vi "Init.vi"(8 "error in (no error)":errorcluster, 10 "CONTROLLER":refnum<class "CONTROLLER.lvclass">, 11 "VIEW in":refnum<class "VIEW.lvclass">) -> (0 "error out":errorcluster, 3 "VIEW out":refnum<class "VIEW.lvclass">)   [LabVIEW 2013, in "VIEW.lvclass"]
uses:
  VIEW.lvclass
  Controller/base/CONTROLLER.lvclass
  VIEW.lvclass/VIEW.ctl
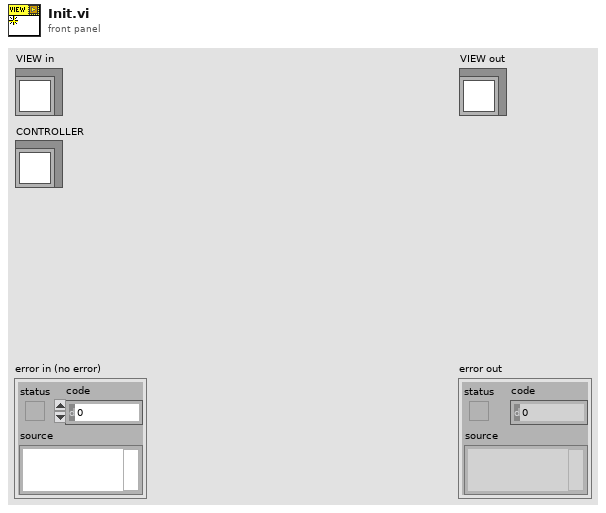
[diagram p1: front panel]
types:
  T1 = cluster{"CtlRef":refnum<vi>, "Name":string, "ClassName":string}
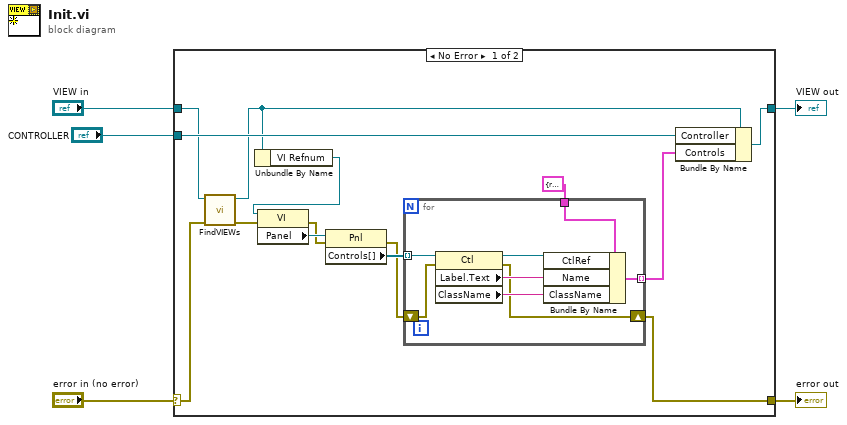
[diagram p0: block diagram]
diagram:
  n1 = case shown="No Error" "error in (no error)" {
    selector: "error in (no error)" -> [w10 w29]
    tunnel: [w13 w29] -> w4
    tunnel: [w12 w28] -> w2
    tunnel: "VIEW in" -> [w8 w28]
    tunnel: "CONTROLLER" -> [w11 _]
    frame No Error {
      n2 = call-dynamic "FindVIEWs.vi"("error in (no error)"=w10, "VIEW in"=w8) -> ("error out"=w9:errorcluster, "VIEW out"=w7:refnum<class "VIEW.lvclass">)  [unwired: 8 in]
      n3 = Unbundle By Name(w7) -> ("VI Refnum"=w6:refnum<vi>)
      n4 = property class="VI"(reference=w6, error in=w9) -> (error out=w18:errorcluster, "Panel"=w19:refnum<vi>)  [unwired: 1 out]
      n5 = property class="Pnl"(reference=w19, error in=w18) -> (error out=w14:errorcluster, "Controls[]"=w17:refnum<vi>[])  [unwired: 1 out]
      n6 = for {
        tunnel: w17 -> [w27] mode=indexing
        tunnel: T1 {"CtlRef"=refnum, "Name"="", "ClassName"=""} ("CtlInfo") -> [w26]
        tunnel: [w22] -> w15 mode=indexing
        shift-right: [w20] -> w13
        shift-left: w14 -> [w21]
        n7 = property class="Ctl"(reference=w27, error in=w21) -> (reference out=w25:refnum<vi>, error out=w20:errorcluster, "Label.Text"=w24:string, "ClassName"=w23:string)
        n8 = Bundle By Name(cluster=w26, "CtlRef"=w25, "Name"=w24, "ClassName"=w23) -> (w22:T1)
      }
      n9 = Bundle By Name(cluster=w7, "Controller"=w11, "Controls"=w15) -> (w12:refnum<class "VIEW.lvclass">)
    }
    frame Error {
    }
  }
  "error out" <- w4
  "VIEW out" <- w2
